vi "RemoteVI Check Overlay Encode.vi"() -> (4 "labels":string[](array[string]), 6 "expected":string[](array[string]), 8 "actual":string[](array[string]), 10 "failures":i32)   [LabVIEW 2020]
doc: "Test support, generated by tests/caraya/build.py from tests/vectors/frame.json - do not edit. Calls RemoteVI Overlay Encode.vi once per vector: the png fields are hex in the vector and decoded to bytes before the call; the message is compared as lowercase hex. Outputs, one element per vector: labels (the vector's name), expected (rendered from the vector), actual (the VI's result rendered the same way), and failures, the number of vectors whose expected and actual differ."
uses:
  source/RemoteVI.lvlib
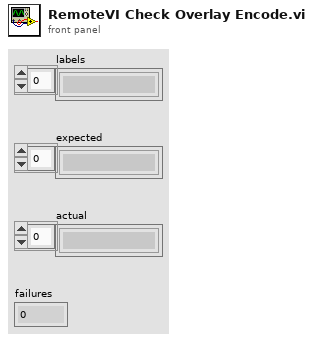
[diagram p1: front panel]
types:
  T1 = cluster{"name":string, "popups":cluster{"x":i16, "y":i16, "png":string}[], "message":string}[]
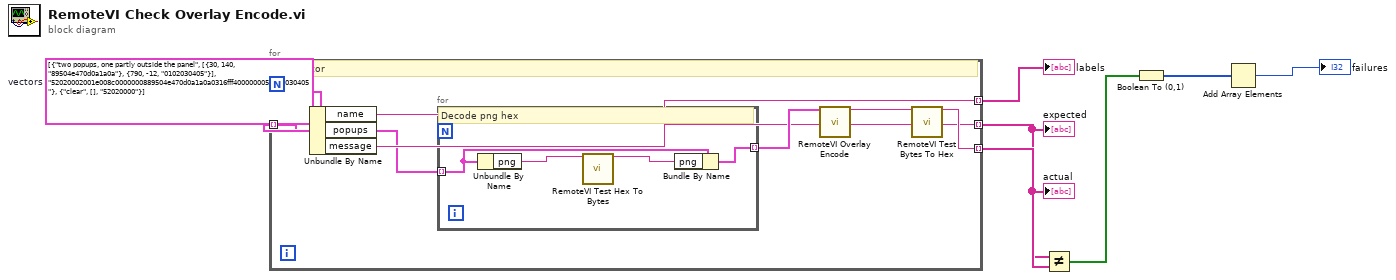
[diagram p0: block diagram]
diagram:
  w1 = T1 [{"name"="two popups, one partly outside the panel", "popups"=[{"x"=30, "y"=140, "png"="89504e470d0a1a0a"}, {"x"=790, "y"=-12, "png"="0102030405"}], "message"="52020002001e008c0000000889504e470d0a1a0a0316fff4000000050102030405"}, {"name"="clear", "popups"=[], "message"="52020000"}]  # vectors
  n1 = for {
    tunnel: w1 -> [w8] mode=indexing
    tunnel: [w9] -> w2 mode=indexing
    tunnel: [w11] -> w3 mode=indexing
    tunnel: [w14] -> w4 mode=indexing
    # "One vector"
    n2 = Unbundle By Name(w8) -> ("name"=w9:string, "popups"=w10:cluster{"x":i16, "y":i16, "png":string}[], "message"=w11:string)
    n3 = for {
      tunnel: w10 -> [w15] mode=indexing
      tunnel: [w18] -> w12 mode=indexing
      # "Decode png hex"
      n4 = Unbundle By Name(w15) -> ("png"=w16:string)
      n5 = call "RemoteVI Test Hex To Bytes.vi"("hex"=w16) -> ("bytes"=w17:string)  [unwired: 14 in]
      n6 = Bundle By Name(cluster=w15, "png"=w17) -> (w18:cluster{"x":i16, "y":i16, "png":string})
    }
    n7 = call "RemoteVI Overlay Encode.vi"("popups"=w12) -> ("message"=w13:string)  [unwired: 14 in]
    n8 = call "RemoteVI Test Bytes To Hex.vi"("bytes"=w13) -> ("hex"=w14:string)  [unwired: 14 in]
  }
  "labels" <- w2
  "expected" <- w3
  "actual" <- w4
  n9 = Not Equal?(x=w3, y=w4) -> (x != y?=w5:bool[])
  n10 = Boolean To (0,1)(Boolean=w5) -> (0, 1=w6:i16[])
  n11 = Add Array Elements(numeric array=w6) -> (sum=→"failures":i16)
